vi "K_S30 F48 init.vi"(8 "error in":errorcluster, 10 "Address":u8=250, 11 "VISA resource":refnum<visa-resource-name>="COM2") -> (0 "error out":errorcluster, 2 "SW-Version":string="5.20-3.52", 3 "Information":T1)   [LabVIEW 2022 SP3]
panel:
  # "Function 48: initialisation of the device\nV1.0, b.v."
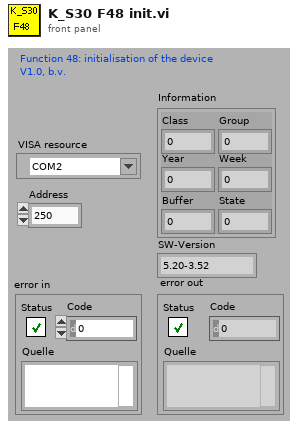
[diagram p1: front panel]
types:
  T1 = cluster{"Class":u8, "Group":u8, "Year":u8, "Week":u8, "Buffer":u8, "State":u8}
  T2 = cluster{"[0]":u8, "[1]":u8, "[2]":u8, "[3]":u8, "[4]":u8, "[5]":u8}
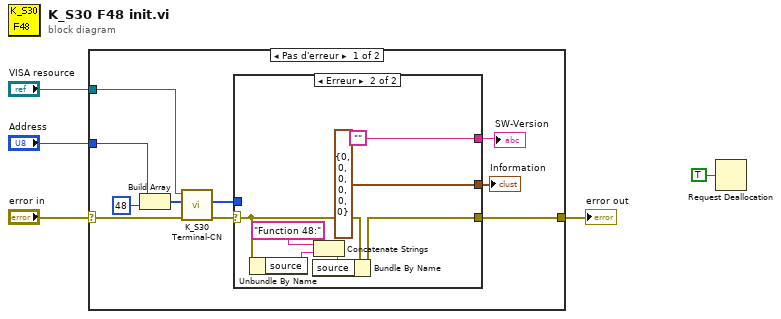
[diagram p0: block diagram]
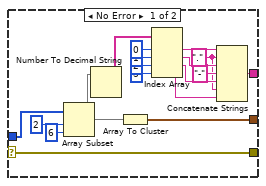
[diagram p2: hidden frame]
diagram:
  n1 = case shown="Pas d'erreur" "error in" {
    selector: "error in" -> [w12 w41]
    tunnel: "Address" -> [w15 _]
    tunnel: [w10 w41] -> w3
    tunnel: "VISA resource" -> [w6 _]
    frame No Error {
      n2 = Build Array(w15, u8 48 ("Element")) -> (w13:u8[])
      n3 = call "K_S30 Terminal-CN.vi"("error in"=w12, "request"=w13, "VISA resource"=w6) -> ("error out"=w11:errorcluster, "response"=w9:u8[])  [unwired: 7 in]
      n4 = case shown="Erreur" w11 {
        selector: w11 -> [w32 w40]
        tunnel: [w32 w38] -> w10
        tunnel: w9 -> [w24 _]
        tunnel: [w33 cluster{u8, u8, u8, u8, u8, u8} {0, 0, 0, 0, 0, 0} ("response")] -> w8
        tunnel: [w16 ""] -> w7
        frame No Error {
          w21 = "." ("String")
          n5 = Array Subset(array=w24, index=2 ("Index"), length=6 ("Länge")) -> (w29:u8[])
          n6 = Number To Decimal String(number=w29) -> (decimal integer string=w23:string[])  [unwired: 1 in]
          n7 = Array To Cluster(array=w29) -> (cluster=w33:T2)
          n8 = Index Array(array=w23, index #1=0 ("Index"), index #2=1 ("Index"), index #3=2 ("Index"), index #4=3 ("Index")) -> (element #1=w22:string, element #2=w28:string, element #3=w26:string, element #4=w25:string)
          n9 = Concatenate Strings(w22, w21, w28, "-" ("String"), w26, w21, w25) -> (w16:string)
        }
        frame Error {
          n10 = Unbundle By Name(w40) -> ("source"=w35:string)
          n11 = Concatenate Strings("Function 48:" ("String"), w35) -> (w39:string)
          n12 = Bundle By Name(cluster=w40, "source"=w39) -> (w38:errorcluster)
        }
      }
      "SW-Version" <- w7
      "Information" <- w8
    }
    frame Error {
    }
  }
  "error out" <- w3
  n13 = Request Deallocation(TRUE ("flag")) -> ()
